vi "select 8000A NR Target.vi"(8 "error in (no error)":errorcluster, 11 "NR in":refnum<class "NR.lvclass">) -> (0 "error out":errorcluster, 3 "NR out":refnum<class "NR.lvclass">)   [LabVIEW 2023, in "ANRITSU Call Box.lvlib" / "NR.lvclass"]
uses:
  NR.lvclass
  NR.lvclass/NR.ctl
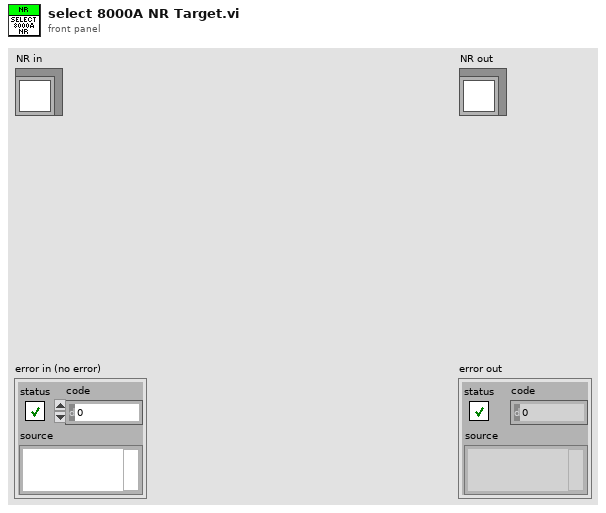
[diagram p1: front panel]
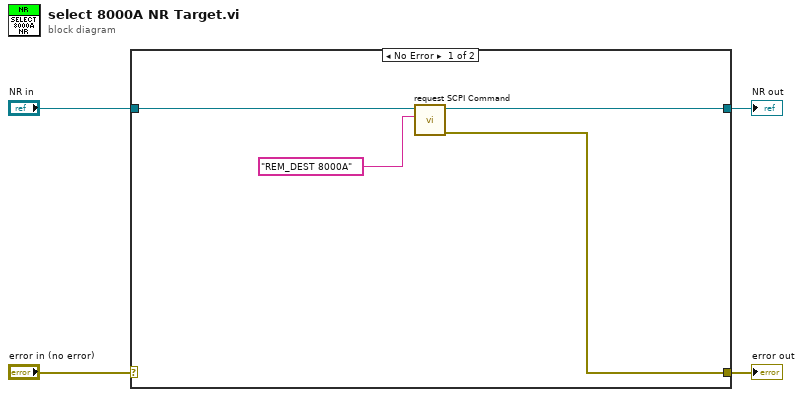
[diagram p0: block diagram]
diagram:
  n1 = case shown="No Error" "error in (no error)" {
    selector: "error in (no error)" -> [_ w10]
    tunnel: [w5 w10] -> w3
    tunnel: [w6 w9] -> w1
    tunnel: "NR in" -> [w8 w9]
    frame No Error {
      n2 = call "request SCPI Command.vi"("SCPI Command"="REM_DEST 8000A" ("write buffer"), "NR in"=w8) -> ("error out"=w5:errorcluster, "NR out"=w6:refnum<class "NR.lvclass">)  [unwired: 8 in]
    }
    frame Error {
    }
  }
  "error out" <- w3
  "NR out" <- w1
